vi "Read Inputs.vi"(8 "error in (no error)":errorcluster, 11 "Modbus in":refnum<class "Modbus.lvclass">) -> (0 "error out":errorcluster, 3 "Modbus out":refnum<class "Modbus.lvclass">)   [LabVIEW 2026, in "Modbus.lvlib" / "Modbus.lvclass"]
uses:
  Modbus.lvclass
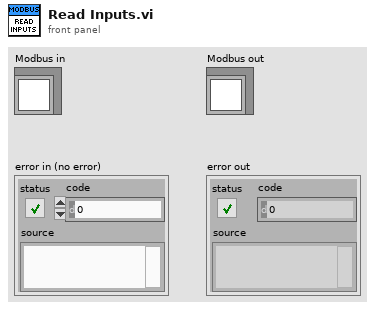
[diagram p1: front panel]
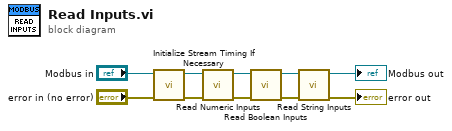
[diagram p0: block diagram]
diagram:
  n1 = call "Initialize Stream Timing If Necessary.vi"("error in (no error)"="error in (no error)", "Modbus in"="Modbus in") -> ("error out"=w1:errorcluster, "Modbus out"=w2:refnum<class "Modbus.lvclass">)  [unwired: 8 in]
  n2 = call "Read Numeric Inputs.vi"("error in (no error)"=w1, "Modbus in"=w2) -> ("error out"=w6:errorcluster, "Modbus out"=w5:refnum<class "Modbus.lvclass">)  [unwired: 8 in]
  n3 = call "Read Boolean Inputs.vi"("error in (no error)"=w6, "Modbus in"=w5) -> ("error out"=w8:errorcluster, "Modbus out"=w7:refnum<class "Modbus.lvclass">)  [unwired: 8 in]
  n4 = call "Read String Inputs.vi"("error in (no error)"=w8, "Modbus in"=w7) -> ("error out"=→"error out":errorcluster, "Modbus out"=→"Modbus out":refnum<class "Modbus.lvclass">)  [unwired: 8 in]
